vi "Read from Hardware.vi"(8 "error in":errorcluster, 10 "Values in":dbl[](array[numeric]), 11 "Ballard ARINC-429 Rx Execution Unit in":refnum<class "Rx Execution Unit.lvclass">) -> (0 "error out":errorcluster, 2 "Values out":dbl[](array[numeric]), 3 "Ballard ARINC-429 Rx Execution Unit out":refnum<class "Rx Execution Unit.lvclass">)   [LabVIEW 2023, in "Ballard ARINC 429 Engine.lvlib" / "Implementation.lvlib" / "Rx Execution Unit.lvclass"]
uses:
  Rx Execution Unit.lvclass
  Rx Execution Unit.lvclass/Rx Execution Unit.ctl
  Execution Unit/Execution Unit.lvclass
  Custom Device/Custom Device.lvlib
  Word.ctl
  Implementation.lvlib
  Logging/Word Logging/Word Logging.lvlib
  Hardware API/Ballard ARINC 429 Hardware API.lvlib
  C:/dev/niveristand-ballard-arinc429-custom-device/Source/Custom Device Support/Engine/Implementation/Execution Unit/Execution Unit.lvclass
  C:/dev/niveristand-ballard-arinc429-custom-device/Source/Custom Device Support/Engine/Interfaces/Execution Unit/Execution Unit.lvclass
  C:/dev/niveristand-ballard-arinc429-custom-device/Source/Custom Device Support/Engine/Implementation/Rx Execution Unit/Rx Execution Unit.lvclass
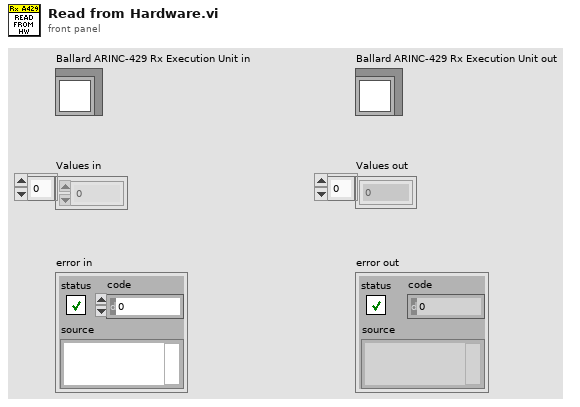
[diagram p1: front panel]
types:
  T1 = cluster{"message info":u32, "data word":u32, "timestamp":dbl}
  T2 = typedef "Ballard ARINC 429 Engine.lvlib/Implementation.lvlib/Word.ctl" = cluster{"message info":cluster{"hardware channel":u8, "label":u8, "SDI":u8}, "data word":u32, "time stamp":dbl}
  T3 = typedef "Ballard ARINC 429 Engine.lvlib/Custom Device.lvlib/Hardware Handles.ctl" = cluster{"core handle":u64, "core reader handle":u64, "channel handles":u64[]}
  T4 = cluster{"gap":i16, "parity":i16, "long word":i16, "bit timing":i16, "timeout":i16}
  T5 = typedef "RT Hardware Channel Settings.ctl" = cluster{"channel #":u16, "channel handle":u64, "labels settings for RT":T6[]}
  T6 = typedef "RT Label Settings.ctl" = cluster{"Name":string, "xmlName":string, "label":T7, "transfer period":u32, "SDI_Enabled":bool, "SDI":u8, "parameter driver data":T8, "transfer type":T12, "has timestamp?":bool, "Label Disable/Trigger Channel Reference":T11, "Message Handle":u64, "Initialized?":bool, "Word Initial Raw Value":u32, "Label Timestamp Channel Data Reference":T13, "disabled":bool}
  T7 = typedef "Label.ctl" = u8
  T8 = typedef "RT Parameters.ctl" = cluster{"parameter definitions":T9[], "Tx parameter refs":T11[]}
  T9 = typedef "Parameter Definition.ctl" = cluster{"start index":i32, "size":i32, "encoding":T10, "signed":bool, "scale multiplier":dbl, "scale offset":dbl}
  T10 = typedef "Encoding and Decoding.lvlib/Encoding.ctl" = enum16{"BNR", "BCD", "Discrete"}
  T11 = typedef "Custom Device API.lvlib/Custom Device Item Ref.ctl" = u64
  T12 = typedef "Transfer Type.ctl" = enum16{"Scheduled", "Acyclic", "Block", "Strobe"}
  T13 = typedef "Custom Device API.lvlib/Data Reference.ctl" = i32
  T14 = typedef "Map of Identifiers to Indexes.ctl" = map{u32, cluster{"channel index":i32, "label index":i32, "start index":i32, "parameters":i32, "timestamp index":i32}}
  T15 = typedef "Rx Channel Data Offsets.ctl" = cluster{"error counts":u32, "rx execution time":i64}
  T16 = cluster{"message info":u32, "data word":u32, "timestamp":dbl}[]
  T17 = typedef "BTICardLV.lvlib/429 Record.ctl" = cluster{"type":u16, "count":u16, "timestamp":u32, "msgact":u16, "decgap":u16, "data":u32, "timestamph":u32}
  T18 = cluster{"gap":bool, "parity":bool, "long word":bool, "bit timing":bool, "timeout":bool}
  T19 = cluster{"hardware channel":u8, "label":u8, "SDI":u8}
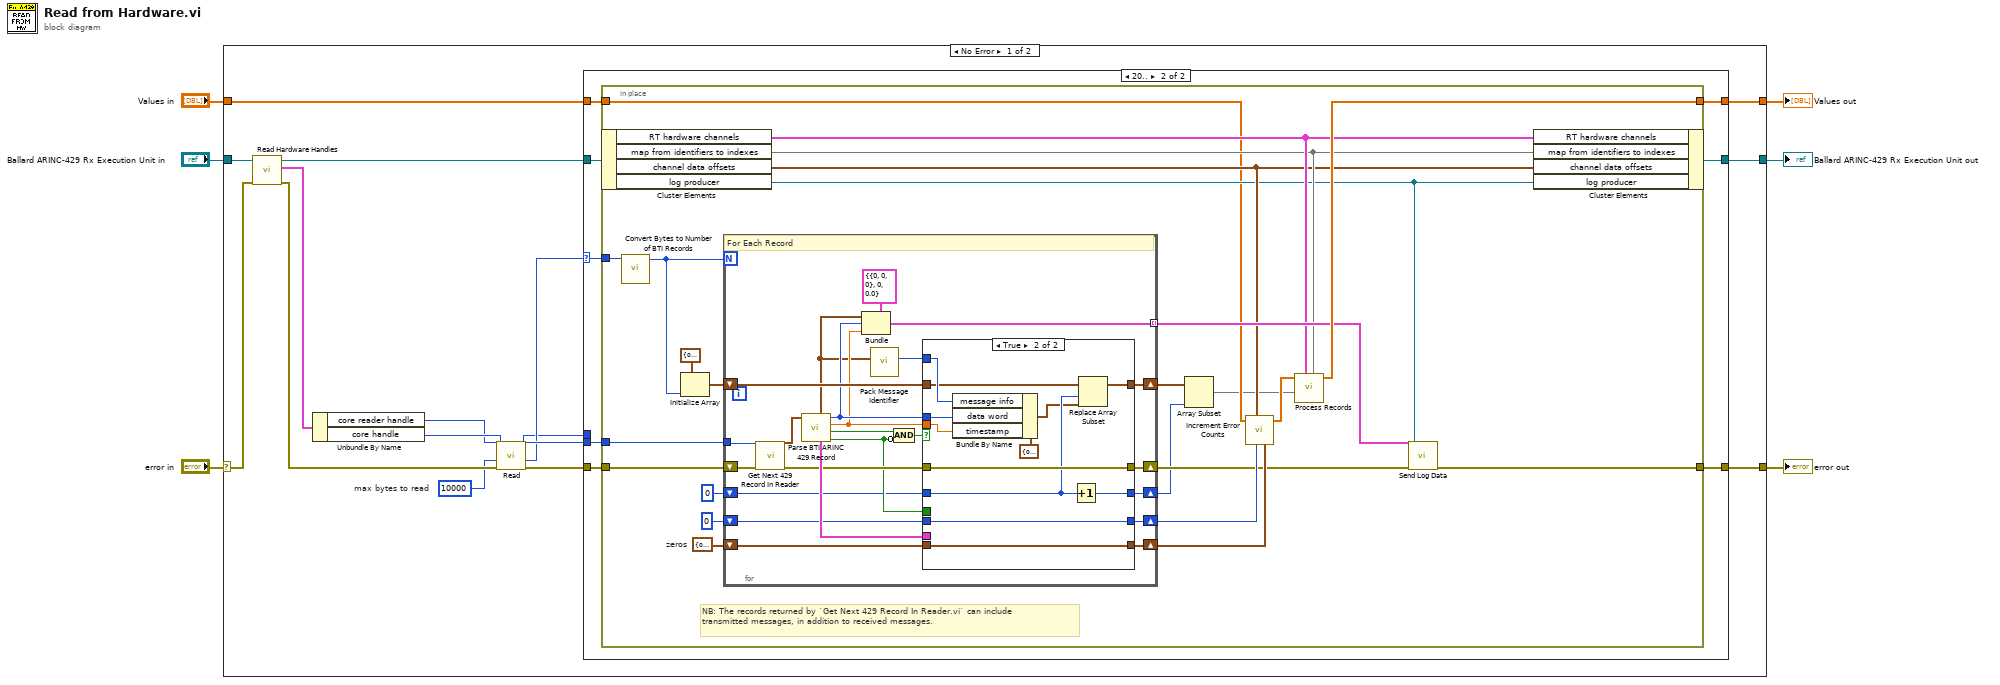
[diagram p0: block diagram]
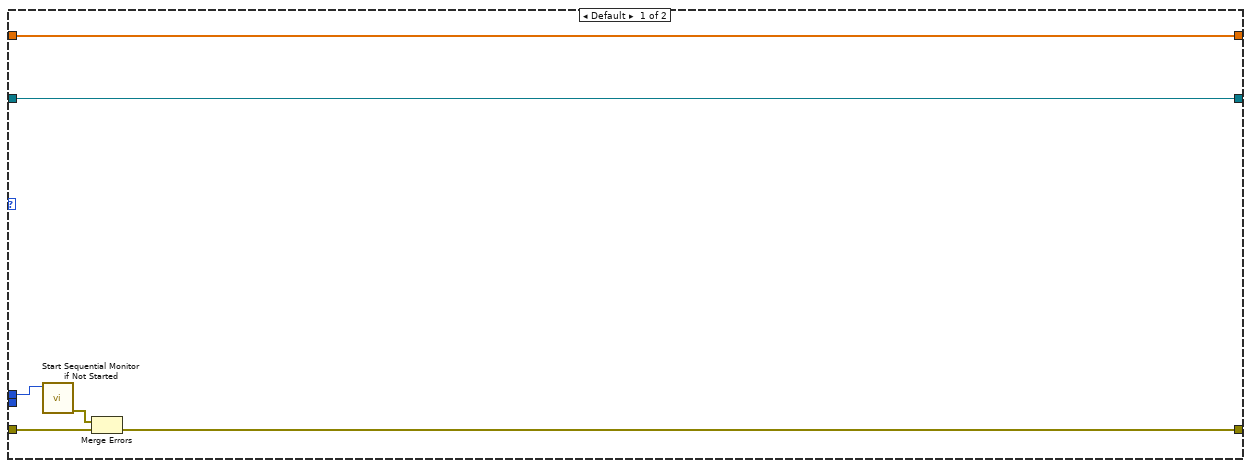
[diagram p2: hidden frame]
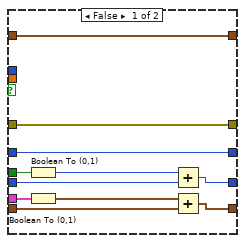
[diagram p3: hidden frame]
diagram:
  n1 = case shown="No Error" "error in" {
    selector: "error in" -> [w22 w108]
    tunnel: [w12 w109] -> w5
    tunnel: "Ballard ARINC-429 Rx Execution Unit in" -> [w21 w109]
    tunnel: [w11 w108] -> w3
    tunnel: [w10 w107] -> w2
    tunnel: "Values in" -> [w9 w107]
    frame No Error {
      w16 = 10000  # max bytes to read
      n2 = call "Read Hardware Handles.vi"("error in"=w22, "Ballard ARINC-429 Execution Unit in"=w21) -> ("error out"=w18:errorcluster, "hardware handles"=w20:T3, "Ballard ARINC-429 Execution Unit out"=w13:refnum<class "Rx Execution Unit.lvclass">)  [unwired: 7 in]
      n3 = Unbundle By Name(w20) -> ("core reader handle"=w17:u64, "core handle"=w19:u64)
      n4 = call "Read.vi"("error in (no error)"=w18, "max bytes to read"=w16, "core reader handle in"=w17, "core handle in"=w19) -> ("error out"=w14:errorcluster, "bytes read"=w8:i32, "core reader handle out"=w15:u64, "core handle out"=w7:u64)  [unwired: 4 in]
      n5 = case shown="20.." w8 {
        selector: w8 -> [_ w29]
        tunnel: w15 -> [_ w36]
        tunnel: w14 -> [w23 w35]
        tunnel: w13 -> [w28 w31]
        tunnel: [w28 w30] -> w12
        tunnel: [w25 w32] -> w11
        tunnel: [w27 w34] -> w10
        tunnel: w9 -> [w27 w33]
        tunnel: w7 -> [w26 _]
        frame Default {
          n6 = call "Start Sequential Monitor if Not Started.vi"("core handle in"=w26) -> ("error out"=w24:errorcluster)  [unwired: 9 in, 1 out]
          n7 = Merge Errors(w24, w23) -> (w25:errorcluster)
        }
        frame 20.. {
          n8 = in-place {
            in-place-border: w36 -> [w60]
            in-place-border: w35 -> [w59]
            in-place-border: [w58] -> w34
            in-place-border: w33 -> [w45]
            in-place-border: [w52] -> w32
            in-place-border: w29 -> [w46]
            w57 = T4 {"gap"=0, "parity"=0, "long word"=0, "bit timing"=0, "timeout"=0}  # zeros
            # "NB: The records returned by `Get Next 429 Record In Reader.vi` can include transmitted messages, in addition to received messages."
            n9 = in-place-cluster #1(w31) -> ("RT hardware channels"=w51:T5[], "map from identifiers to indexes"=w50:T14, "channel data offsets"=w49:T15, "log producer"=w48:refnum<class "Log Producer.lvclass">)
            n10 = call "Convert Bytes to Number of BTI Records.vi"("bytes read"=w46) -> ("number of records read"=w43:i32)  [unwired: 10 in]
            n11 = Initialize Array(T1 {"message info"=0, "data word"=0, "timestamp"=0.0}, w43) -> (w41:T16)
            n12 = for {
              N: w43 -> [_]
              tunnel: w60 -> [w83]
              shift-right: [w72] -> w47
              shift-left: w59 -> [w82]
              shift-right: [w78] -> w54
              shift-left: w57 -> [w77]
              shift-right: [w70] -> w55
              shift-left: i16 0 -> [w69]
              tunnel: [w65] -> w53 mode=indexing
              shift-right: [w62] -> w37
              shift-left: 0 -> [w63]
              shift-right: [w80] -> w39
              shift-left: w41 -> [w79]
              # "For Each Record"
              n13 = call "Get Next 429 Record In Reader.vi"("error in (no error)"=w82, "core reader handle in"=w83) -> ("error out"=w73:errorcluster, "record out"=w81:T17)  [unwired: 7 in, 1 out]
              n14 = call "Parse BTI ARINC 429 Record.vi"("record"=w81) -> ("receiving error"=w71:bool, "hit"=w75:bool, "time stamp"=w66:dbl, "data word"=w67:u32, "specific errors"=w76:T18, "message info"=w64:T19)  [unwired: 5 in]
              n15 = Bundle(cluster=T2 {"message info"={"hardware channel"=0, "label"=0, "SDI"=0}, "data word"=0, "time stamp"=0.0} ("Word"), "message info"=w64, "data word"=w67, "time stamp"=w66) -> (w65:T2)
              n16 = call "Pack Message Identifier.vi"("message identifiers"=w64) -> ("packed message identifier"=w61:u32)  [unwired: 10 in]
              n17 = Compound Arithmetic op=AND(w75, invert w71) -> (w74:bool)
              n18 = case shown="True" w74 {
                tunnel: w67 -> [_ w100]
                tunnel: [w94 w95] -> w80
                tunnel: w79 -> [w94 w96]
                tunnel: w77 -> [w92 w106]
                tunnel: [w88 w106] -> w78
                tunnel: w66 -> [_ w99]
                tunnel: w76 -> [w91 _]
                tunnel: w73 -> [w90 w105]
                tunnel: [w90 w105] -> w72
                tunnel: w71 -> [w89 _]
                tunnel: [w87 w104] -> w70
                tunnel: w69 -> [w85 w104]
                tunnel: w61 -> [_ w101]
                tunnel: w63 -> [w84 w98]
                tunnel: [w84 w103] -> w62
                frame False {
                  n19 = Boolean To (0,1)(Boolean=w89) -> (0, 1=w86:i16)
                  n20 = Boolean To (0,1)(Boolean=w91) -> (0, 1=w93:T4)
                  n21 = Add(x=w86, y=w85) -> (x+y=w87:i16)
                  n22 = Add(x=w93, y=w92) -> (x+y=w88:T4)
                }
                frame True {
                  n23 = Bundle By Name(cluster=T1 {"message info"=0, "data word"=0, "timestamp"=0.0}, "message info"=w101, "data word"=w100, "timestamp"=w99) -> (w97:T1)
                  n24 = Increment(x=w98) -> (x+1=w103:i32)
                  n25 = Replace Array Subset(array=w96, new element=w97, index=w98) -> (w95:T16)
                }
              }
            }
            n26 = Array Subset(array=w39, length=w37) -> (w38:T16)  [unwired: 1 in]
            n27 = call "Increment Error Counts.vi"("specific errors"=w54, "receiving errors"=w55, "channel data offsets"=w49, "values in"=w45) -> ("values out"=w44:dbl[])  [unwired: 7 in]
            n28 = call "Process Records.vi"("map from message info to indexes"=w50, "RT hardware channel data"=w51, "map of message info to data word"=w38, "parameter values in"=w44) -> ("parameter values out"=w58:dbl[])  [unwired: 4 in, 1 out]
            n29 = call "Send Log Data.vi"("error in (no error)"=w47, "Data"=w53, "Producer in"=w48) -> ("error out"=w52:errorcluster)  [unwired: 7 in, 1 out]
            n30 = in-place-cluster #1("RT hardware channels"=w51, "map from identifiers to indexes"=w50, "channel data offsets"=w49, "log producer"=w48) -> (w30:refnum<class "Rx Execution Unit.lvclass">)
          }
        }
      }
    }
    frame Error {
    }
  }
  "error out" <- w3
  "Ballard ARINC-429 Rx Execution Unit out" <- w5
  "Values out" <- w2
